vi "VIH HelpGen - Palette - Get Palette Items (method 2).vi"(8 "error in":errorcluster, 11 "Palette Path":path) -> (0 "error out":errorcluster, 2 "Items Array":T1[](array[typedef]), 3 "dup Palette Path":path)   [LabVIEW 2014]
doc: "::: VI Helpeks :::\nCopyright (c) 2000-2026 Konstantin Shifershteyn. All rights reserved."
uses:
  VIH HelpGen Typedef - Palette - Item Info Cluster.ctl
  VIH HelpGen Typedef - Palette - Item Type Enum.ctl
panel:
  # "VI Helpeks\nCopyright (c) 2012-2026 Konstantin Shifershteyn"
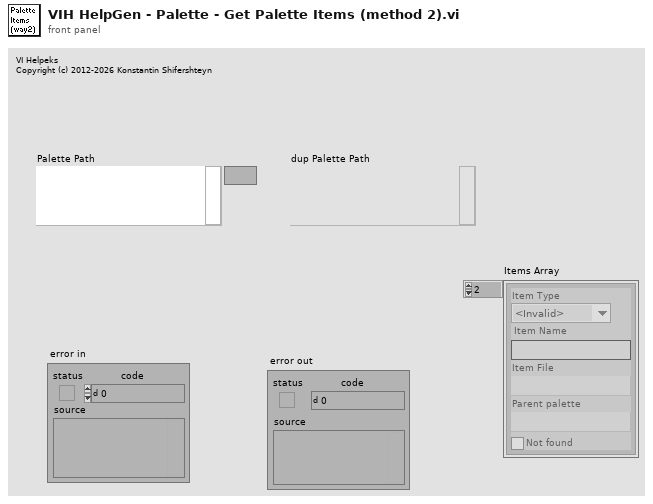
[diagram p1: front panel]
types:
  T1 = typedef "VIH HelpGen Typedef - Palette - Item Info Cluster.ctl" = cluster{"Item Type":T2, "Item Name":string, "Item File":path, "Parent palette":path, "Not found":bool}
  T2 = typedef "VIH HelpGen Typedef - Palette - Item Type Enum.ctl" = enum32{"<Invalid>", "<unknown>", "VI", "Menu", "LV Func", "Express VI", "Poly VI", "CTL", "HTML"}
  T3 = cluster{"Palette Item Type":enum32{"Submenu", "VI", "Express VI", "Built In", "Empty"}, "short name":string, "Item name":string, "file path":path, "image":u8[]}[]
  T4 = enum32{"Submenu", "VI", "Express VI", "Built In", "Empty"}
  T5 = typedef "Palette Menu.lvlib/Palette Data.ctl" = cluster{"display name":string, "view format":T6, "palette width":i16, "items":T7, "256 color icon":picture, "B&W color icon":picture, "help information":T9, "palette description":string, "synchronize information":T10}
  T6 = typedef "Palette Menu.lvlib/View Format.ctl" = u16
  T7 = typedef "Palette Menu.lvlib/Items.ctl" = T8[]
  T8 = typedef "Palette Menu.lvlib/Item.ctl" = cluster{"item path":path, "library path (.lvlib)":path, "use default lvlib palette":bool, "short name":string, "place VI contents":bool, "hide synchronized item":bool, "reserve spot for synch item":bool, "configure when placing VI contents":bool}
  T9 = typedef "Palette Menu.lvlib/Help Info.ctl" = cluster{"help tag":string, "help file path ":path}
  T10 = typedef "Palette Menu.lvlib/Synchronize Info.ctl" = cluster{"synchronize with directory":bool, "synchronize directory path":path}
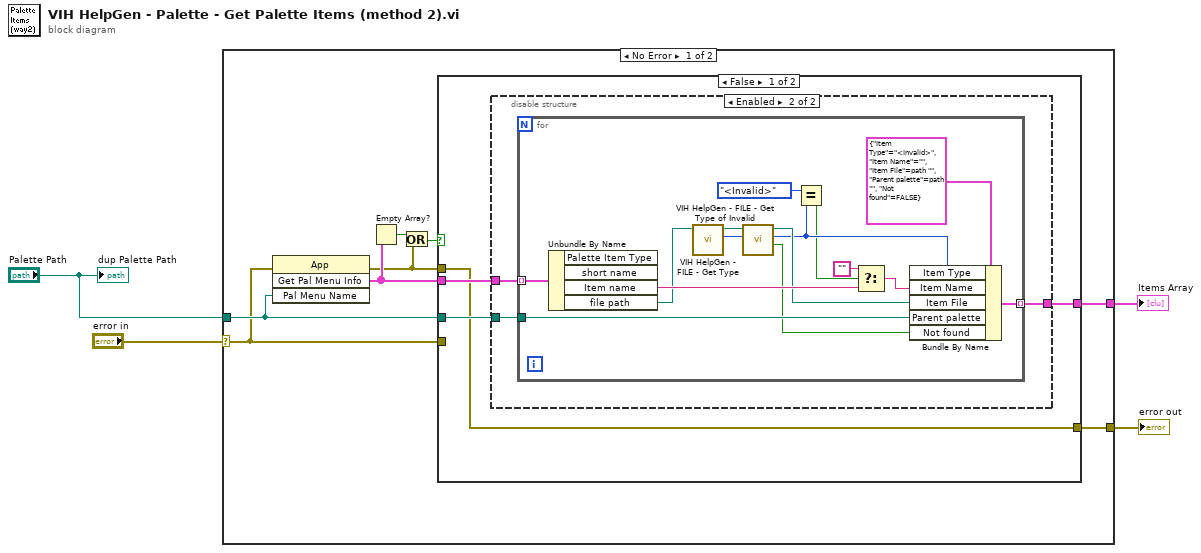
[diagram p0: block diagram]
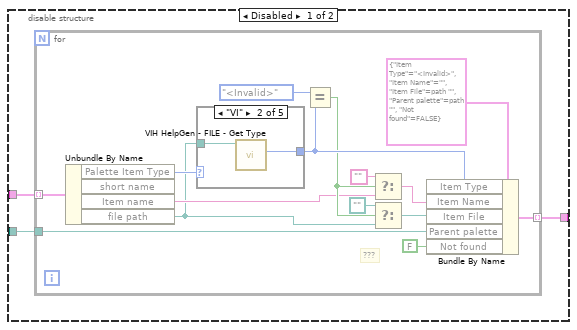
[diagram p2: hidden frame]
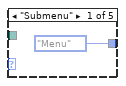
[diagram p3: hidden frame]
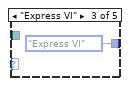
[diagram p4: hidden frame]
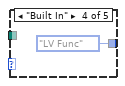
[diagram p5: hidden frame]
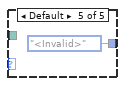
[diagram p6: hidden frame]
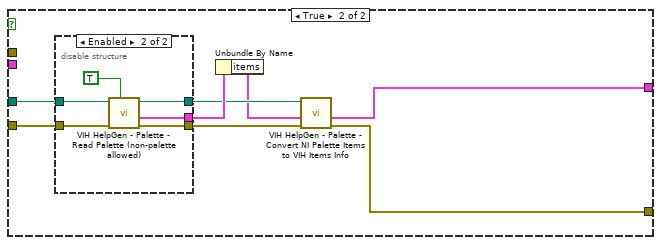
[diagram p7: hidden frame]
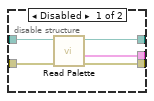
[diagram p8: hidden frame]
diagram:
  n1 = case shown="No Error" "error in" {
    selector: "error in" -> [w9 w78]
    tunnel: "Palette Path" -> [w12 _]
    tunnel: [w11 _] -> w2
    tunnel: [w10 w78] -> w1
    frame No Error {
      n2 = invoke class="App" method="Get Pal Menu Info"(error in=w9, "Pal Menu Name"=w12) -> (error out=w6:errorcluster, "Get Palette Menu Info"=w8:T3)  [unwired: 2 in, 2 out]
      n3 = Empty Array?(array=w8) -> (empty?=w7:bool)
      n4 = Or(x=w7, y=w6) -> (x .or. y?=w5:bool)
      n5 = case shown="False" w5 {
        tunnel: w8 -> [w16 _]
        tunnel: w12 -> [w15 w66]
        tunnel: [w14 w61] -> w11
        tunnel: [w13 w59] -> w10
        tunnel: w9 -> [_ w64]
        tunnel: w6 -> [w13 _]
        frame False {
          n6 = disable-structure shown="Enabled" {
            disable-tunnel: w16 -> [w19 w43]
            disable-tunnel: w15 -> [w18 w42]
            disable-tunnel: [w17 w41] -> w14
            frame Disabled {
              n7 = for {
                tunnel: w19 -> [w34] mode=indexing
                tunnel: w18 -> [w33]
                tunnel: [w31] -> w17 mode=indexing
                # "???"
                n8 = Unbundle By Name(w34) -> ("Palette Item Type"=w32:T4, "Item name"=w27:string, "file path"=w26:path)  [unwired: 1 out]
                n9 = case shown="\"VI\"" w32 {
                  tunnel: [VIH_HelpGen_Typedef_-_Palette_-_Item_Type_Enum."Menu" ("Item Type") w36 VIH_HelpGen_Typedef_-_Palette_-_Item_Type_Enum."Express VI" ("Item Type") VIH_HelpGen_Typedef_-_Palette_-_Item_Type_Enum."LV Func" ("Item Type") VIH_HelpGen_Typedef_-_Palette_-_Item_Type_Enum."<Invalid>" ("Item Type")] -> w30
                  tunnel: w26 -> [_ w37 _ _ _]
                  frame "Submenu" {
                  }
                  frame "VI" {
                    n10 = call "VIH HelpGen - FILE - Get Type.vi"("File Path"=w37) -> ("File Type"=w36:T2)  [unwired: 8 in, 2 out]
                  }
                  frame "Express VI" {
                  }
                  frame "Built In" {
                  }
                  frame Default {
                  }
                }
                n11 = Equal?(x=VIH_HelpGen_Typedef_-_Palette_-_Item_Type_Enum."<Invalid>", y=w30) -> (x = y?=w28:bool)
                n12 = Select(t="", s=w28, f=w27) -> (s? t:f=w24:string)
                n13 = Select(t=path "", s=w28, f=w26) -> (s? t:f=w25:path)
                n14 = Bundle By Name(cluster=T1 {"Item Type"=enum."<Invalid>", "Item Name"="", "Item File"=path "", "Parent palette"=path "", "Not found"=FALSE} ("Item Info"), "Item Type"=w30, "Item Name"=w24, "Item File"=w25, "Parent palette"=w33, "Not found"=FALSE) -> (w31:T1)
              }
            }
            frame Enabled {
              n15 = for {
                tunnel: w43 -> [w58] mode=indexing
                tunnel: w42 -> [w57]
                tunnel: [w56] -> w41 mode=indexing
                n16 = Unbundle By Name(w58) -> ("Item name"=w55:string, "file path"=w51:path)  [unwired: 2 out]
                n17 = call "VIH HelpGen - FILE - Get Type.vi"("File Path"=w51) -> ("File Type"=w49:T2, "dup File Path"=w50:path)  [unwired: 8 in, 1 out]
                n18 = call "VIH HelpGen - FILE - Get Type of Invalid.vi"("File Type"=w49, "File Path"=w50) -> ("Not found"=w47:bool, "File Type out"=w45:T2, "File Path out"=w48:path)  [unwired: 6 in, 1 out]
                n19 = Equal?(x=VIH_HelpGen_Typedef_-_Palette_-_Item_Type_Enum."<Invalid>", y=w45) -> (x = y?=w44:bool)
                n20 = Select(t="", s=w44, f=w55) -> (s? t:f=w54:string)
                n21 = Bundle By Name(cluster=T1 {"Item Type"=enum."<Invalid>", "Item Name"="", "Item File"=path "", "Parent palette"=path "", "Not found"=FALSE} ("Item Info"), "Item Type"=w45, "Item Name"=w54, "Item File"=w48, "Parent palette"=w57, "Not found"=w47) -> (w56:T1)
              }
            }
          }
        }
        frame True {
          n22 = disable-structure shown="Enabled" {
            disable-tunnel: w66 -> [w71 w77]
            disable-tunnel: [w70 w74] -> w65
            disable-tunnel: w64 -> [w69 w76]
            disable-tunnel: [w68 w75] -> w63
            disable-tunnel: [w67 w73] -> w60
            frame Disabled {
              n23 = call <vilib>:"Read Palette.vi"("error in (no error)"=w69, "palette path"=w71) -> ("error out"=w67:errorcluster, "palette data"=w70:T5, "duplicate palette path"=w68:path)  [unwired: 7 in]
            }
            frame Enabled {
              n24 = call "VIH HelpGen - Palette - Read Palette (non-palette allowed).vi"("Get Items (F)"=TRUE, "error in"=w76, "Palette Path"=w77) -> ("error out"=w73:errorcluster, "palette data"=w74:T5, "dup Palette Menu Path"=w75:path)  [unwired: 6 in]
            }
          }
          n25 = Unbundle By Name(w65) -> ("items"=w62:T7)
          n26 = call "VIH HelpGen - Palette - Convert NI Palette Items to VIH Items Info.vi"("error in"=w60, "Palette Items"=w62, "Palette Path"=w63) -> ("error out"=w59:errorcluster, "Items Array"=w61:T1[])  [unwired: 6 in, 1 out]
        }
      }
    }
    frame Error {
    }
  }
  "Items Array" <- w2
  "error out" <- w1
  "dup Palette Path" <- "Palette Path"
